vi "[ce] ODE Solver.vi"(4 "parameters":cluster{"name":string, "value":dbl}[](array[cluster]) {"value" format="%.2f"}, 5 "method (R-K)":enum16{"Runge Kutta", "Euler"}(ring), 6 "time":string="t", 7 "h (step rate)":dbl=0.1 format="%.4f", 8 "error in":errorcluster, 9 "equation descriptions":T1(array[cluster]) {"init value" format="%.2f"}, 10 "time end":dbl=1.0 format="%.2f", 11 "time start":dbl format="%.2f") -> (0 "error out":errorcluster, 1 "ticks":u32, 2 "X Values (solution)":dbl[][](array[numeric]) format="%.2f", 3 "Times":dbl[](array[numeric]) format="%.2f")   [LabVIEW 2021]
doc: "This VI solves ordinary differential equations:\n dX(t)/dt = F(X,t) , X(0) = X0\nIn addition, the VI allows specifying additional parameters and evaluating them in formula.\nTo determine the solution you can use either Runge-Kutta or Euler method. The Runge Kutta method is more accurate, the Euler method is faster.\n\n::: CalcExpress Toolkit :::\nCopyright (c) 2000-2026 Konstantin Shifershteyn. All rights reserved."
panel:
  # "dX(t)/dt = F(X,t) , X(0)=X0"
  # "Example:\n\n time start: 0.0 \n time end: 1.0\n h: 0.1\n time: t\n equation descriptions:\n 1)  ------\n    variable:   x\n    formula:    sin(t*x)+y\n    init value: 1.0\n 2)  ------\n    variable:   y\n    formula:    x-y\n    init value: 1.0"
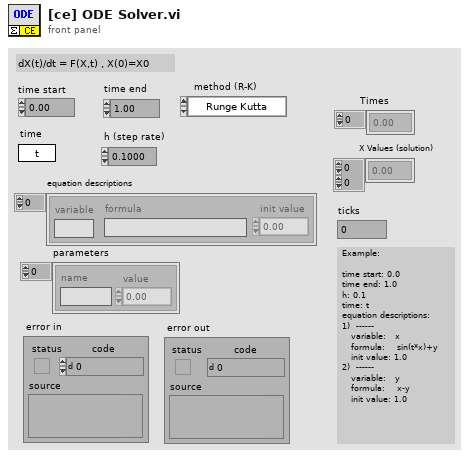
[diagram p1: front panel]
types:
  T1 = cluster{"variable":string, "formula":string, "init value":dbl}[]
  T2 = typedef "VarMan Variable Context Handle.ctl" = i32
  T3 = typedef "CalcExpress Instance RefNum.ctl" = refnum<k1>
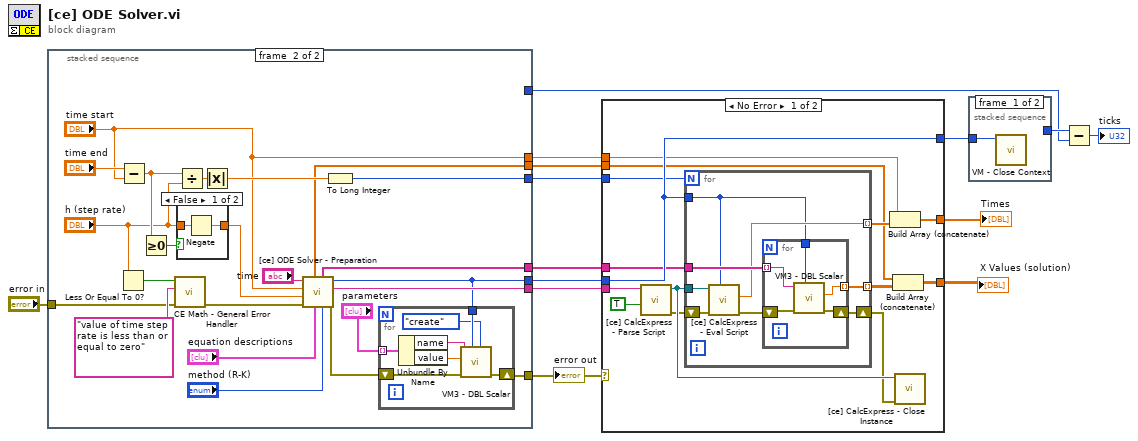
[diagram p0: block diagram]
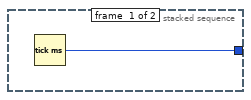
[diagram p2: hidden frame]
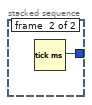
[diagram p4: hidden frame]
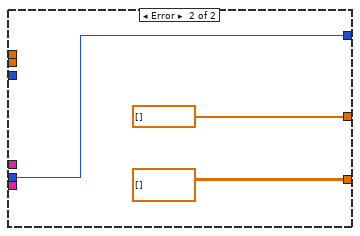
[diagram p5: hidden frame]
diagram:
  n1 = stacked-sequence {
    tunnel: [w15 _] -> w12
    tunnel: [_ w18] -> w9
    tunnel: [_ w38] -> w8
    tunnel: [_ w26] -> w6
    tunnel: [_ w16] -> w1
    tunnel: [_ w28] -> w5
    tunnel: [_ "time start"] -> w4
    tunnel: "error in" -> [_ w27]
    tunnel: [_ w20] -> w2
    frame #0 {
      n2 = Tick Count (ms)() -> (millisecond timer value=w15:u32)
    }
    frame #1 {
      n3 = Less Or Equal To 0?(x="h (step rate)") -> (x <= 0?=w36:bool)
      n4 = Subtract(x="time end", y="time start") -> (x-y=w32:dbl)
      n5 = Greater Or Equal To 0?(x=w32) -> (x >= 0?=w31:bool)
      n6 = call "CE Math - General Error Handler.vi"("error before"=w27, "message"="value of time step rate is less than or equal to zero", "error? (T)"=w36) -> ("error out"=w37:errorcluster)  [unwired: 5 in, 1 out]
      n7 = Divide(x=w32, y="h (step rate)") -> (x/y=w33:dbl)
      n8 = case shown="False" w31 {
        tunnel: "h (step rate)" -> [w47 w48]
        tunnel: [w46 w48] -> w21
        frame False {
          n9 = Negate(x=w47) -> (-x=w46:dbl)
        }
        frame True {
        }
      }
      n10 = Absolute Value(x=w33) -> (abs(x)=w30:dbl)
      n11 = call "[ce] ODE Solver - Preparation.vi"("method"="method (R-K)", "equation parameters"="equation descriptions", "error in"=w37, "h value"=w21, "time value"="time start", "time"="time") -> ("error out"=w17:errorcluster, "expression"=w38:string, "VC Handle"=w18:T2, "var names"=w26:string[], "X0"=w20:dbl[])  [unwired: 1 in]
      n12 = To Long Integer(number=w30) -> (32bit integer=w28:i32)
      n13 = for {
        shift-right: [w42] -> w16
        shift-left: w17 -> [w43]
        tunnel: "parameters" -> [w41] mode=indexing
        tunnel: w18 -> [w40]
        n14 = Unbundle By Name(w41) -> ("name"=w44:string, "value"=w45:dbl)
        n15 = call "VM3 - DBL Scalar.vi"("cmd (read)"=enum16{"create", "destroy", "write", "read"}."create", "VC Handle"=w40, "error in"=w43, "value in"=w45, "name_spec"=w44) -> ("error out"=w42:errorcluster)  [unwired: 3 in, 3 out]
      }
    }
  }
  "error out" <- w1
  n16 = case shown="No Error" w1 {
    tunnel: [w58 dbl[] []] -> w11
    tunnel: [w56 dbl[][] []] -> w10
    tunnel: w9 -> [w60 w78]
    tunnel: w8 -> [w53 _]
    tunnel: [w60 w78] -> w7
    tunnel: w6 -> [w59 _]
    tunnel: w4 -> [w57 _]
    tunnel: w5 -> [w55 _]
    tunnel: w2 -> [w54 _]
    frame No Error {
      n17 = call "[ce] CalcExpress - Parse Script.vi"("create instance"=TRUE, "expression"=w53) -> ("error out"=w50:errorcluster, "CE InstanceRef"=w52:T3)  [unwired: 4 in, 2 out]
      n18 = for {
        N: w55 -> [_]
        shift-right: [w68] -> w49
        shift-left: w50 -> [w65]
        tunnel: [w67] -> w62 mode=indexing
        tunnel: [w70] -> w61 mode=indexing
        tunnel: w60 -> [w63]
        tunnel: w59 -> [w69]
        tunnel: w52 -> [w64]
        n19 = call "[ce] CalcExpress - Eval Script.vi"("VC Handle"=w63, "error in"=w65, "CE InstanceRef"=w64) -> ("error out"=w66:errorcluster, "numeric value"=w67:dbl)  [unwired: 2 in, 3 out]
        n20 = for {
          shift-right: [w73] -> w68
          shift-left: w66 -> [w74]
          tunnel: w69 -> [w75] mode=indexing
          tunnel: w63 -> [w72]
          tunnel: [w71] -> w70 mode=indexing
          n21 = call "VM3 - DBL Scalar.vi"("VC Handle"=w72, "error in"=w74, "name_spec"=w75) -> ("error out"=w73:errorcluster, "value out"=w71:dbl)  [unwired: 5 in, 2 out]
        }
      }
      n22 = Build Array (concatenate)(w57, w62) -> (w58:dbl[])
      n23 = Build Array (concatenate)(w54, w61) -> (w56:dbl[][])
      n24 = call "[ce] CalcExpress - Close Instance.vi"("error in"=w49, "CE InstanceRef"=w52) -> ()  [unwired: 5 in, 3 out]
    }
    frame Error {
    }
  }
  "Times" <- w11
  "X Values (solution)" <- w10
  n25 = stacked-sequence {
    tunnel: [_ w80] -> w14
    tunnel: w7 -> [w79 _]
    frame #0 {
      n26 = call "VM - Close Context.vi"("VC Handle"=w79) -> ()  [unwired: 9 in, 2 out]
    }
    frame #1 {
      n27 = Tick Count (ms)() -> (millisecond timer value=w80:u32)
    }
  }
  n28 = Subtract(x=w14, y=w12) -> (x-y=→"ticks":u32)
